vi "UDP Simulation.vi"() -> ()   [LabVIEW 2023]
panel:
  out "Same data count":i32
  in  "Stop on Timeout":bool
  out "Read Loop Timer":u32
  in  "Read Timeout":i32=1000
  out "Timeout":bool
  in  "Write?":bool
  in  "Port Write (Remote)":u16=5000
  in  "IP Write (Remote)":string="192.168.1.69"
  out "IP Read (Remote)":string
  in  "Data Write":string="\u0001\u0002\u0003\u0004\u0005\u0006\u0007\b"
  in  "Port Read (Local)":u16=60002
  out "Data received":string
  out "Port Read (Remote)":u16
  in  "Port Write (Local)":u16=60001
  in  "IP (Local)":string="192.168.1.107"
  in  "stop":bool
  out "Read":errorcluster
  out "Write":errorcluster
  out "Write Close":errorcluster
  out "Read Close":errorcluster
  # "Write"
  # "Read"
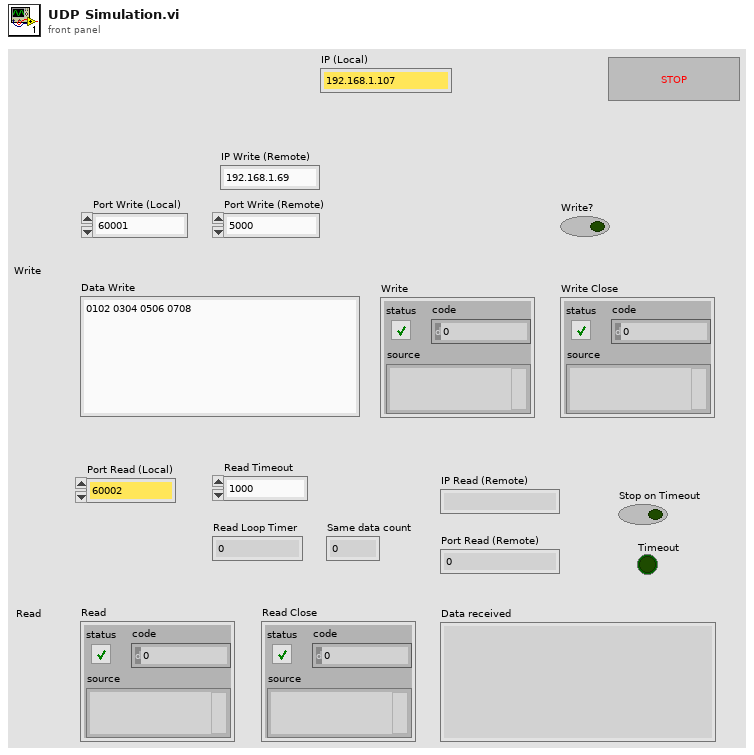
[diagram p1: front panel]
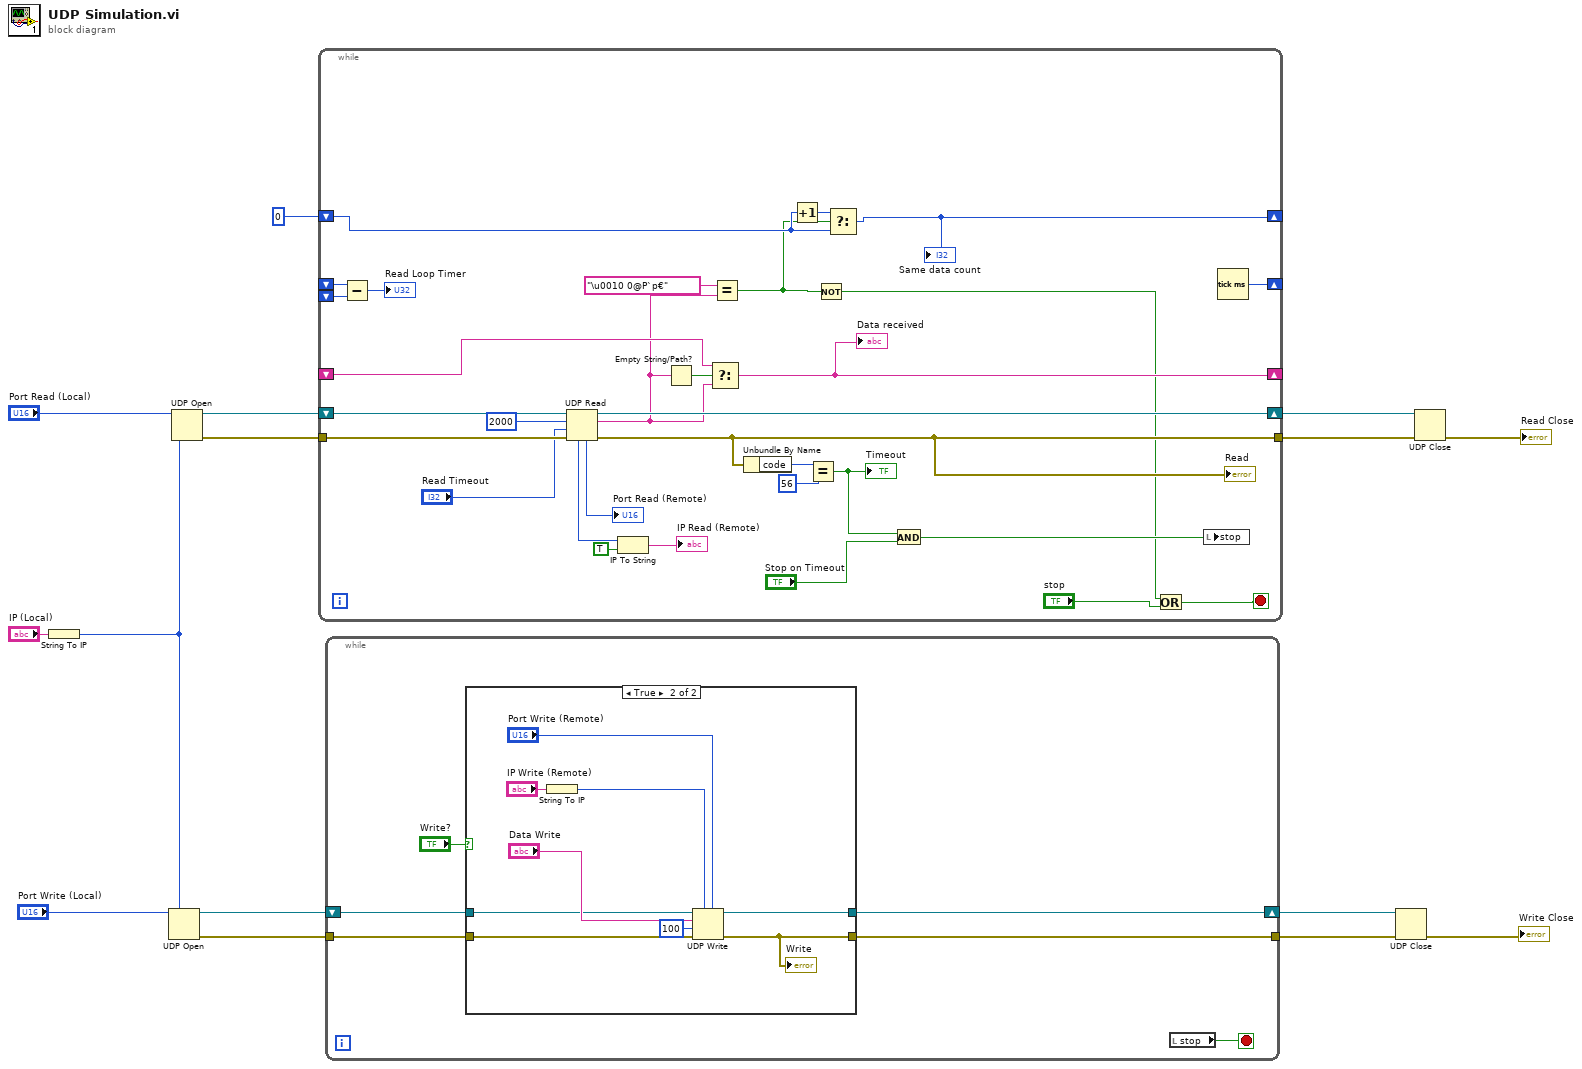
[diagram p0: block diagram]
diagram:
  n1 = String To IP(1:"IP (Local)") -> (0:w6:u32)
  n2 = UDP Open(7:w6, 11:"Port Write (Local)") -> (port=w3:refnum<k16>, 0:w10:errorcluster)  [unwired: 3 in, 1 out]
  n3 = UDP Open(7:w6, 11:"Port Read (Local)") -> (port=w13:refnum<k16>, 0:w15:errorcluster)  [unwired: 3 in, 1 out]
  n4 = while {
    shift-right: [w44] -> w12
    shift-left: w13 -> [w45]
    tunnel: w15 -> [w46]
    tunnel: [w37] -> w14
    shift-right: [w33] -> _
    shift-left: _ -> [w25]
    shift-right: [w32] -> _
    shift-left: _ -> [w30]
    shift-left: _ -> [w31]
    shift-right: [w22] -> _
    shift-left: 0 -> [w23]
    stop <- w19 stop-if-true
    n5 = Subtract(x=w30, y=w31) -> (x-y=→"Read Loop Timer":u32)
    n6 = UDP Read(connection ID=w45, max size (548)=2000, timeout ms (25000)="Read Timeout", 8:w46) -> (data out=w21:string, error out=w37:errorcluster, 3:w44:refnum<k16>, 4:→"Port Read (Remote)":u16, 6:w39:u32)
    "Read" <- w37
    n7 = IP To String(1:TRUE ("dot notation? (F)"), 2:w39) -> (0:→"IP Read (Remote)":string)
    n8 = Empty String/Path?(string/path=w21) -> (empty?=w34:bool)
    n9 = Select(t=w25, s=w34, f=w21) -> (s? t:f=w33:string)
    "Data received" <- w33
    n10 = Equal?(x="\u0010 0@P`p€", y=w21) -> (x = y?=w17:bool)
    n11 = Unbundle By Name(w37) -> ("code"=w36:i32)
    n12 = Increment(x=w23) -> (x+1=w24:i32)
    n13 = Equal?(x=w36, y=56) -> (x = y?=w27:bool)
    "Timeout" <- w27
    n14 = Not(x=w17) -> (.not. x?=w16:bool)
    n15 = Select(t=w24, s=w17, f=w23) -> (s? t:f=w22:i32)
    "Same data count" <- w22
    n16 = And(x=w27, y="Stop on Timeout") -> (x .and. y?=w28:bool)
    n17 = Or(x=w16, y="stop") -> (x .or. y?=w19:bool)
    n18 = local write "stop"(w28) -> ()
    n19 = Tick Count (ms)() -> (millisecond timer value=w32:u32)
  }
  n20 = while {
    tunnel: w10 -> [w52]
    tunnel: [w51] -> w9
    shift-right: [w48] -> w2
    shift-left: w3 -> [w49]
    stop <- w50 stop-if-true
    n21 = case shown="True" "Write?" {
      tunnel: w52 -> [w54 w63]
      tunnel: [w54 w62] -> w51
      tunnel: w49 -> [w53 w59]
      tunnel: [w53 w58] -> w48
      frame False {
      }
      frame True {
        n22 = String To IP(1:"IP Write (Remote)") -> (0:w56:u32)
        n23 = UDP Write(address=w56, port or service name="Port Write (Remote)", connection ID=w59, data in="Data Write", 8:w63, 9:100 ("timeout ms (25000)")) -> (error out=w62:errorcluster, 3:w58:refnum<k16>)
        "Write" <- w62
      }
    }
    n24 = local read "stop"() -> (w50:bool)
  }
  n25 = UDP Close(connection ID=w2, 8:w9) -> (error out=→"Write Close":errorcluster)  [unwired: 1 out]
  n26 = UDP Close(connection ID=w12, 8:w14) -> (error out=→"Read Close":errorcluster)  [unwired: 1 out]
